vi "Read TopVI Tag.vi"(8 "error in":errorcluster, 9 "Alias":string, 10 "Project Reference":refnum<vi>) -> (0 "error out":errorcluster, 2 "TopVI Tag":string, 3 "TopVI Path":path)   [LabVIEW 2020]
doc: "Reads the TopVI tag from the program and returns the tag value and the path to the VI the tag points to."
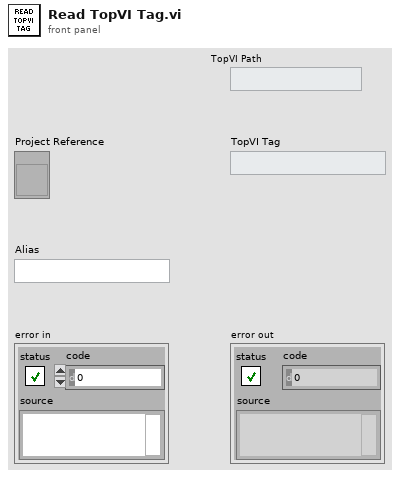
[diagram p1: front panel]
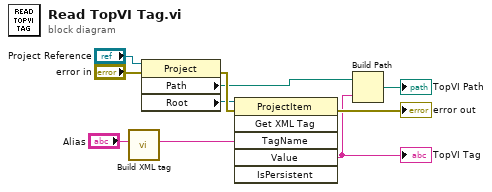
[diagram p0: block diagram]
diagram:
  n1 = call "Build XML tag.vi"("Alias"="Alias") -> ("XML Tag"=w2:string)  [unwired: 10 in]
  n2 = property class="Project"(reference="Project Reference", error in="error in") -> (error out=w10:errorcluster, "Path"=w6:path, "Root"=w5:refnum<vi>)  [unwired: 1 out]
  n3 = invoke class="ProjectItem" method="Get XML Tag"(reference=w5, error in=w10, "TagName"=w2) -> (error out=→"error out":errorcluster, "Value"=w4:string)  [unwired: 3 in, 4 out]
  "TopVI Tag" <- w4
  n4 = Build Path(base path=w6, name or relative path=w4) -> (appended path=→"TopVI Path":path)
